vi "AlliGator Get XY Graph Refnum by Name.vi"(8 "error in (no error)":errorcluster, 11 "XY Graph Name":string) -> (0 "error out":errorcluster, 3 "XY Graph reference":T1)   [LabVIEW 2021, in "AlliGator GUI.lvlib"]
doc: "Returns a reference to one of the Graph objects in AlliGator based on the provided <B>XY Graph Name</B>.."
uses:
  AlliGator GUI.lvlib
  Graphs/XY Graph/XY Graph Refnum.ctl
  <vilib>/Utility/error.llb/Error Cluster From Error Code.vi
  <vilib>/ErrorRing/Error Ring.xnode
  Strings/Strings.lvlib
  Decay Graph/AlliGator Decay Graph.lvlib
  Decay Statistics/AlliGator Decay Statistics.lvlib
  Intensity Time Trace/AlliGator Intensity Time Trace.lvlib
  Phasor Ratio/AlliGator Phasor Ratio.lvlib
  Lifetime & Other Parameters/AlliGator Lifetime & Other Parameters.lvlib
  Graphs/XY Graph/XY Graph Add-Ons.lvlib
panel:
  # "see the AlliGator License on the block diagram (Ctrl+E or Window:Show Block Diagram)"
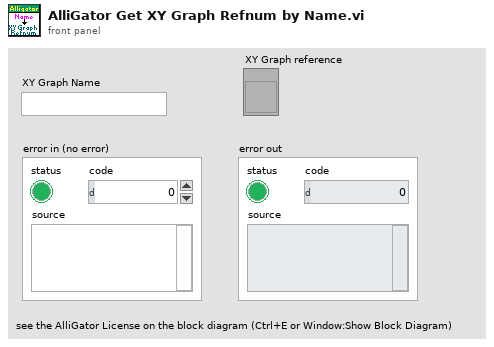
[diagram p1: front panel]
types:
  T1 = typedef "XY Graph Add-Ons.lvlib/XY Graph Refnum.ctl" = refnum<vi>
  T2 = typedef "AlliGator Decay Graph.lvlib/AlliGator Decay Graph Ctrl Refnums.ctl" = cluster{"Decay Graph":refnum<vi>, "Decay Graph Active":refnum<vi>}
  T3 = typedef "AlliGator Decay Statistics.lvlib/AlliGator Decay Statistics Graph Ctrl Refnums.ctl" = cluster{"Decay Statistics Graph":refnum<vi>, "Decay Statistics Bin":refnum<vi>}
  T4 = typedef "AlliGator Intensity Time Trace.lvlib/AlliGator Intensity Time Trace Ctrl Refnums.ctl" = cluster{"Intensity Time Trace":refnum<vi>, "Time Step":refnum<vi>, "Use File Timestamp":refnum<vi>}
  T5 = typedef "AlliGator Phasor Ratio.lvlib/AlliGator Phasor Ratio Graph Ctrl Refnums.ctl" = cluster{"Phasor Ratio Graph":refnum<vi>}
  T6 = typedef "AlliGator Lifetime & Other Parameters.lvlib/AlliGator Lifetime & Other Parameters Ctrl Refnums.ctl" = cluster{"Lifetime Graph":refnum<vi>}
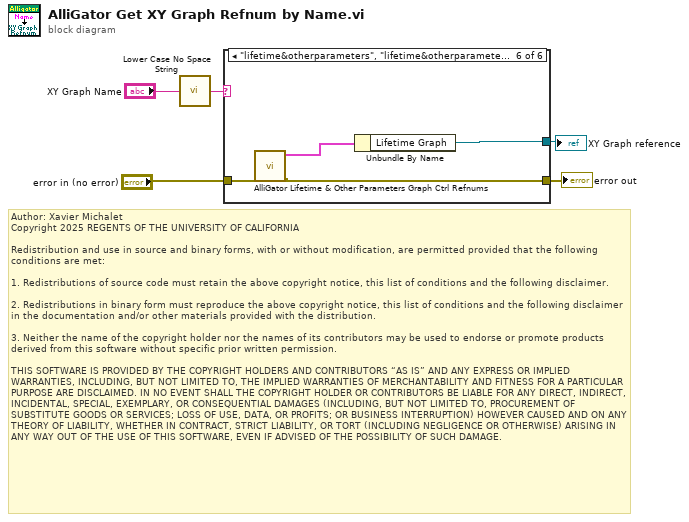
[diagram p0: block diagram]
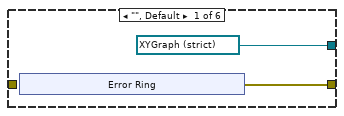
[diagram p2: hidden frame]
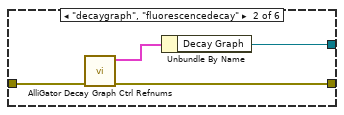
[diagram p3: hidden frame]
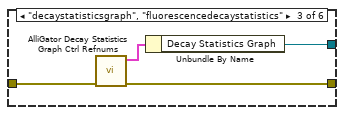
[diagram p4: hidden frame]
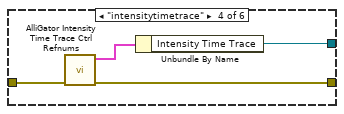
[diagram p5: hidden frame]
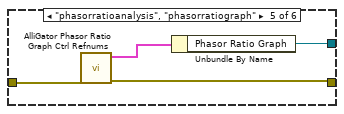
[diagram p6: hidden frame]
diagram:
  # "Author: Xavier Michalet\nCopyright 2025 REGENTS OF THE UNIVERSITY OF CALIFORNIA\n\nRedistribution and use in source and binary forms, with or without modification, are permitted provided that the following conditions are met:\n\n1. Redistributions of source code must retain the above copyright notice, this list of conditions and the following disclaimer.\n\n2. Redistributions in binary form must reproduce the above copyright notice, this list of conditions and the following disclaimer in the documentation and/or other materials provided with the distribution.\n\n3. Neither the name of the copyright holder nor the names of its contributors may be used to endorse or promote products derived from this software without specific prior written permission.\n\nTHIS SOFTWARE IS PROVIDED BY THE COPYRIGHT HOLDERS AND CONTRIBUTORS “AS IS” AND ANY EXPRESS OR IMPLIED WARRANTIES, INCLUDING, BUT NOT LIMITED TO, THE IMPLIED WARRANTIES OF MERCHANTABILITY AND FITNESS FOR A PARTICULAR PURPOSE ARE DISCLAIMED. IN NO EVENT SHALL THE COPYRIGHT HOLDER OR CONTRIBUTORS BE LIABLE FOR ANY DIRECT, INDIRECT, INCIDENTAL, SPECIAL, EXEMPLARY, OR CONSEQUENTIAL DAMAGES (INCLUDING, BUT NOT LIMITED TO, PROCUREMENT OF SUBSTITUTE GOODS OR SERVICES; LOSS OF USE, DATA, OR PROFITS; OR BUSINESS INTERRUPTION) HOWEVER CAUSED AND ON ANY THEORY OF LIABILITY, WHETHER IN CONTRACT, STRICT LIABILITY, OR TORT (INCLUDING NEGLIGENCE OR OTHERWISE) ARISING IN ANY WAY OUT OF THE USE OF THIS SOFTWARE, EVEN IF ADVISED OF THE POSSIBILITY OF SUCH DAMAGE."
  n1 = call "Lower Case No Space String.vi"("String"="XY Graph Name") -> ("Lower Case No Space String"=w4:string)
  n2 = case shown="\"lifetime&otherparameters\", \"lifetime&otherparametersgraph\", \"lifetimegraph\"" w4 {
    tunnel: [refnum<vi> refnum ("Decay Graph") w13 w16 w20 w27 w31] -> w3
    tunnel: [w7 w12 w18 w22 w25 w29] -> w2
    tunnel: "error in (no error)" -> [_ w15 w19 w23 w26 w30]
    frame "", Default {
      n3 = xnode "Error Ring"() -> ("error out"=w7:errorcluster)
    }
    frame "decaygraph", "fluorescencedecay" {
      n4 = call "AlliGator Decay Graph Ctrl Refnums.vi"("error in (no error)"=w15) -> ("error out"=w12:errorcluster, "Decay Graph Ctrl Refnums"=w14:T2)  [unwired: 9 in]
      n5 = Unbundle By Name(w14) -> ("Decay Graph"=w13:refnum<vi>)
    }
    frame "decaystatisticsgraph", "fluorescencedecaystatistics" {
      n6 = call "AlliGator Decay Statistics Graph Ctrl Refnums.vi"("error in (no error)"=w19) -> ("error out"=w18:errorcluster, "Decay Statistics Graph Ctrl Refnums"=w17:T3)  [unwired: 9 in]
      n7 = Unbundle By Name(w17) -> ("Decay Statistics Graph"=w16:refnum<vi>)
    }
    frame "intensitytimetrace" {
      n8 = call "AlliGator Intensity Time Trace Ctrl Refnums.vi"("error in (no error)"=w23) -> ("error out"=w22:errorcluster, "Intensity Time Trace Ctrl Refnums"=w21:T4)  [unwired: 9 in]
      n9 = Unbundle By Name(w21) -> ("Intensity Time Trace"=w20:refnum<vi>)
    }
    frame "phasorratioanalysis", "phasorratiograph" {
      n10 = call "AlliGator Phasor Ratio Graph Ctrl Refnums.vi"("error in (no error)"=w26) -> ("error out"=w25:errorcluster, "Phasor Ratio Graph Ctrl Refnums"=w24:T5)  [unwired: 9 in]
      n11 = Unbundle By Name(w24) -> ("Phasor Ratio Graph"=w27:refnum<vi>)
    }
    frame "lifetime&otherparameters", "lifetime&otherparametersgraph", "lifetimegraph" {
      n12 = call "AlliGator Lifetime & Other Parameters Graph Ctrl Refnums.vi"("error in (no error)"=w30) -> ("error out"=w29:errorcluster, "Lifetime & Other Parameters Graph Ctrl Refnums"=w28:T6)  [unwired: 9 in]
      n13 = Unbundle By Name(w28) -> ("Lifetime Graph"=w31:refnum<vi>)
    }
  }
  "error out" <- w2
  "XY Graph reference" <- w3
